vi "Remove_User.vi"(8 "error in (no error)":errorcluster) -> (0 "error out":errorcluster)   [LabVIEW 2021]
panel:
  in  "Add User":bool
  in  "Password":string
  in  "User Name":string
  # "REMOVE USER"
  # "Give User Name and Password"
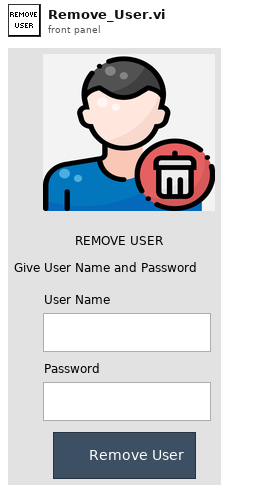
[diagram p1: front panel]
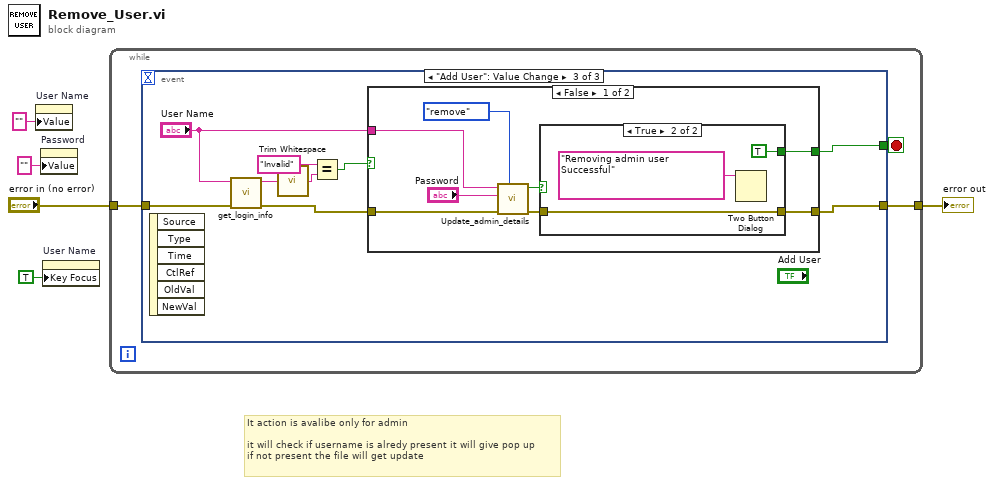
[diagram p0: block diagram]
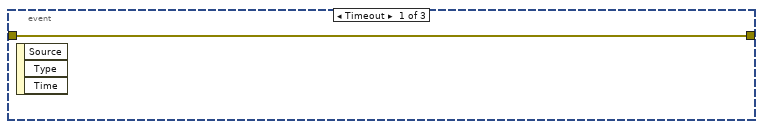
[diagram p2: hidden frame]
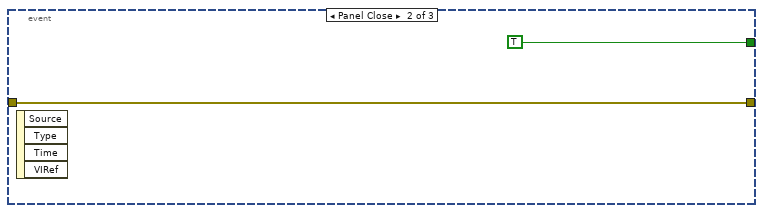
[diagram p3: hidden frame]
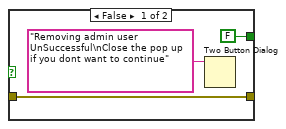
[diagram p4: hidden frame]
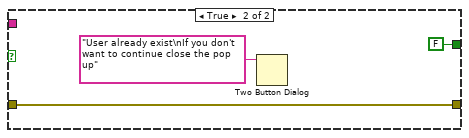
[diagram p5: hidden frame]
diagram:
  # "It action is avalibe only for admin\n\nit will check if username is alredy present it will give pop up\nif not present the file will get update"
  n1 = property on="User Name" class="Str"("Value"="" ("User Name")) -> ()  [unwired: 2 in, 2 out]
  n2 = property on="Password" class="Str"("Value"="" ("Password")) -> ()  [unwired: 2 in, 2 out]
  n3 = property on="User Name" class="Str"("Key Focus"=TRUE) -> ()  [unwired: 2 in, 2 out]
  n4 = while {
    tunnel: "error in (no error)" -> [w7]
    tunnel: [w6] -> w4
    stop <- w8 stop-if-true
    n5 = event shown="[2] \"Add User\": Value Change" {
      selector: _ -> [_ _ _]
      dyn-events: _ -> [_ _ _]
      timeout: _ -> [_ _ _]
      tunnel: [_ TRUE w20] -> w8
      tunnel: w7 -> [w9 w11 w18]
      tunnel: [w9 w11 w19] -> w6
      event Timeout {
        n6 = event-data() -> ()  [unwired: 1 in, 3 out]
      }
      event Panel Close {
        n7 = event-data() -> ()  [unwired: 1 in, 4 out]
      }
      event "Add User": Value Change {
        n8 = event-data() -> ()  [unwired: 1 in, 6 out]
        n9 = call "get_login_info.vi"("error in (no error)"=w18, "User"="User Name") -> ("error out"=w17:errorcluster, "User_name"=w15:string)  [unwired: 7 in, 1 out]
        n10 = call <vilib>:"Trim Whitespace.vi"("string"=w15) -> ("trimmed string"=w12:string)  [unwired: 1 in]
        n11 = Equal?(x="Invalid", y=w12) -> (x = y?=w13:bool)
        n12 = case shown="False" w13 {
          tunnel: [w27 FALSE] -> w20
          tunnel: w17 -> [w26 w35]
          tunnel: [w25 w35] -> w19
          tunnel: "User Name" -> [w23 _]
          frame False {
            n13 = call "Update_admin_details.vi"("Enum"=enum16{"add", "update", "read", "remove"}."remove", "error in (no error)"=w26, "string"="Password", "User"=w23) -> ("error out"=w24:errorcluster, "Status"=w21:bool)  [unwired: 6 in]
            n14 = case shown="True" w21 {
              tunnel: [FALSE TRUE] -> w27
              tunnel: [w29 w32] -> w25
              tunnel: w24 -> [w29 w32]
              frame False {
                n15 = Two Button Dialog(message="Removing admin user UnSuccessful\nClose the pop up if you dont want to continue") -> ()  [unwired: 2 in, 1 out]
              }
              frame True {
                n16 = Two Button Dialog(message="Removing admin user Successful") -> ()  [unwired: 2 in, 1 out]
              }
            }
          }
          frame True {
            n17 = Two Button Dialog(message="User already exist\nIf you don't want to continue close the pop up") -> ()  [unwired: 2 in, 1 out]
          }
        }
      }
    }
  }
  "error out" <- w4
